vi "Read File (Complete).vi"(8 "error in (no error)":errorcluster, 11 "ConfigManager.Text in":refnum<class "ConfigManager.Text.lvclass">) -> (0 "error out":errorcluster, 2 "String":string, 3 "ConfigManager.Text out":refnum<class "ConfigManager.Text.lvclass">)   [LabVIEW 2013, in "CfgManager.Text.lvlib" / "ConfigManager.Text.lvclass"]
uses:
  ConfigManager.Text.lvclass
  Manager/ConfigManager.lvclass/ConfigManager.ctl
  Manager/ConfigManager.lvclass
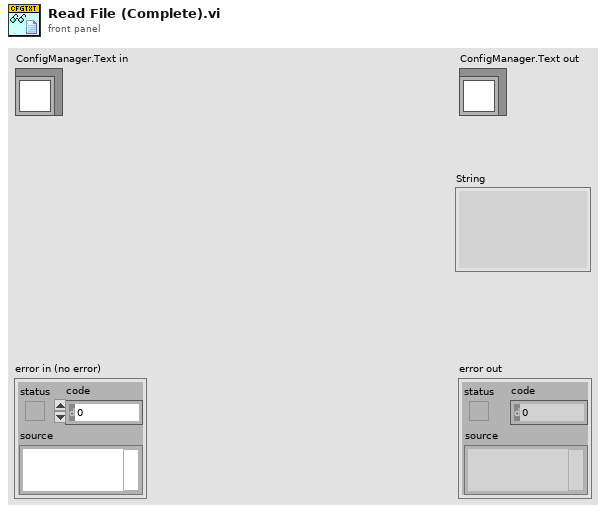
[diagram p1: front panel]
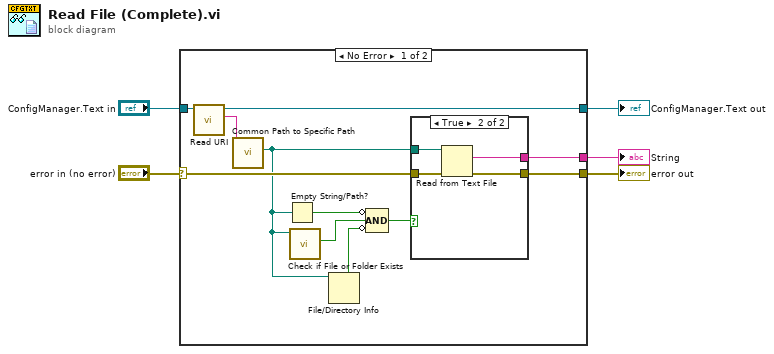
[diagram p0: block diagram]
diagram:
  n1 = case shown="No Error" "error in (no error)" {
    selector: "error in (no error)" -> [w15 w23]
    tunnel: [w14 w23] -> w4
    tunnel: [w7 w22] -> w2
    tunnel: "ConfigManager.Text in" -> [w8 w22]
    tunnel: [w16 _] -> w1
    frame No Error {
      n2 = call "Read URI.vi"("ConfigManager in"=w8) -> ("URI"=w6:string, "ConfigManager out"=w7:refnum<class "ConfigManager.Text.lvclass">)  [unwired: 9 in]
      n3 = call "Common Path to Specific Path.vi"("common path"=w6) -> ("specific path"=w9:path)  [unwired: 10 in]
      n4 = Empty String/Path?(string/path=w9) -> (empty?=w13:bool)
      n5 = call <vilib>:"Check if File or Folder Exists.vi"("path"=w9) -> ("file or folder exists?"=w12:bool)  [unwired: 8 in, 2 out]
      n6 = File/Directory Info(path=w9) -> (directory=w11:bool)  [unwired: 1 in, 6 out]
      n7 = Compound Arithmetic op=AND(invert w13, w12, invert w11) -> (w10:bool)
      n8 = case shown="True" w10 {
        tunnel: [_ w21] -> w16
        tunnel: w15 -> [w17 w20]
        tunnel: [w17 w19] -> w14
        tunnel: w9 -> [_ w18]
        frame False {
        }
        frame True {
          n9 = Read from Text File(file (use dialog)=w18, error in=w20) -> (text=w21:string, error out=w19:errorcluster)  [unwired: 2 in, 2 out]
        }
      }
    }
    frame Error {
    }
  }
  "error out" <- w4
  "ConfigManager.Text out" <- w2
  "String" <- w1
